vi "Jump Back.vi"(8 "error in":errorcluster, 10 "VI Name":string, 11 "Data in":T1={"PeekVI Reference"=refnum, "SubPanel"=refnum, "Peek Stack Tree Ref"=refnum, "Open Button Ref"=refnum, "Top VI"=refnum, "Active VI"=refnum, "Stack"=[], "Last FP State"=enum."Standard"}) -> (0 "error out":errorcluster, 3 "Data out":T1={"PeekVI Reference"=refnum, "SubPanel"=refnum, "Peek Stack Tree Ref"=refnum, "Open Button Ref"=refnum, "Top VI"=refnum, "Active VI"=refnum, "Stack"=[], "Last FP State"=enum."Standard"})   [LabVIEW 2020, in "Peek Window.lvlib"]
uses:
  Peek Window.lvlib
  MHL Data Cluster.ctl
  VI Types/Standard VI Type/Standard VI Type.lvclass
  VI Types/Standard VI Type/Standard VI Type.lvclass/Standard VI Type.ctl
  VI Types/Standard VI Type/Read Full Qualified Name.vi
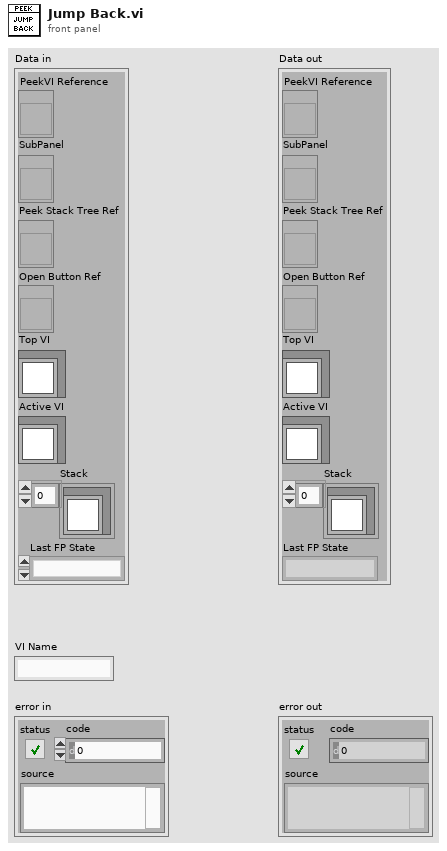
[diagram p1: front panel]
types:
  T1 = typedef "Peek Window.lvlib/MHL Data Cluster.ctl" = cluster{"PeekVI Reference":refnum<vi>, "SubPanel":refnum<vi>, "Peek Stack Tree Ref":refnum<vi>, "Open Button Ref":refnum<vi>, "Top VI":refnum<class "Standard VI Type.lvclass">, "Active VI":refnum<class "Standard VI Type.lvclass">, "Stack":refnum<class "Standard VI Type.lvclass">[], "Last FP State":enum32{"Invalid", "Standard", "Closed", "Hidden", "Minimized", "Maximized"}}
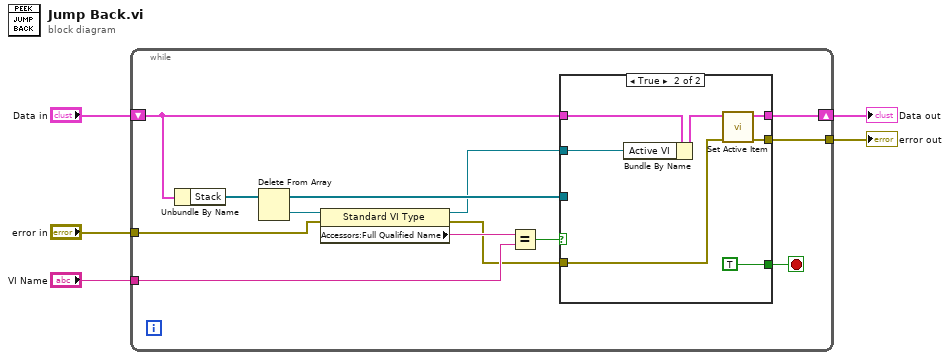
[diagram p0: block diagram]
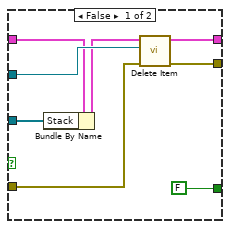
[diagram p2: hidden frame]
diagram:
  n1 = while {
    tunnel: "error in" -> [w6]
    tunnel: [w14] -> w2
    tunnel: "VI Name" -> [w18]
    shift-right: [w16] -> w4
    shift-left: "Data in" -> [w15]
    stop <- w12 stop-if-true
    n2 = Unbundle By Name(w15) -> ("Stack"=w13:refnum<class "Standard VI Type.lvclass">[])
    n3 = Delete From Array(array=w13) -> (deleted portion=w10:refnum<class "Standard VI Type.lvclass">, array with subset deleted=w11:refnum<class "Standard VI Type.lvclass">[])  [unwired: 2 in]
    n4 = property class="Standard VI Type"(reference=w10, error in=w6) -> (reference out=w8:refnum<class "Standard VI Type.lvclass">, error out=w7:errorcluster, "Accessors:Full Qualified Name"=w9:string)
    n5 = Equal?(x=w9, y=w18) -> (x = y?=w17:bool)
    n6 = case shown="True" w17 {
      tunnel: [w21 w32] -> w16
      tunnel: w15 -> [w19 w28]
      tunnel: [w25 w31] -> w14
      tunnel: w7 -> [w26 w30]
      tunnel: w11 -> [w24 _]
      tunnel: [FALSE TRUE] -> w12
      tunnel: w8 -> [w22 w27]
      frame False {
        n7 = Bundle By Name(cluster=w19, "Stack"=w24) -> (w20:T1)
        n8 = call "Delete Item.vi"("error in (no error)"=w26, "Removed VI"=w22, "Data in"=w20) -> ("error out"=w25:errorcluster, "Data out"=w21:T1)  [unwired: 7 in]
      }
      frame True {
        n9 = Bundle By Name(cluster=w28, "Active VI"=w27) -> (w29:T1)
        n10 = call "Set Active Item.vi"("error in (no error)"=w30, "Data Cluster"=w29) -> ("error out"=w31:errorcluster, "Module Data"=w32:T1)  [unwired: 8 in]
      }
    }
  }
  "Data out" <- w4
  "error out" <- w2
